vi "Get VI Inputs and Outputs.vi"   [LabVIEW 2016, in "SLL Application.lvlib"]
doc: "Get the list of controls and indicators of a given VI reference.\n\nIf the VI refnum input is not passed or invalid, it will automatically get the refnum of caller VI and use."
uses:
  SLL Application.lvlib
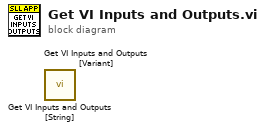
[diagram p0: block diagram]
diagram:
  n1 = call "Get VI Inputs and Outputs [String].vi"() -> ()  [unwired: 8 in, 4 out]
  n2 = call "Get VI Inputs and Outputs [Variant].vi"() -> ()  [unwired: 8 in, 4 out]
